vi "LabVIEW结合知识库调用本地大模型.vi"() -> ()   [LabVIEW 2023, in "LabVIEW RAG.lvlib"]
uses:
  RAG_LV_API/LabVIEW RAG.lvlib
  labview-local-model/openai_message.ctl
  labview-local-model/chat-completion req.ctl
  <vilib>/Utility/error.llb/Trim Whitespace One-Sided.vi
  labview-local-model/LabVIEW LLM.lvlib
  labview-ai-share/LabVIEW AI Base.lvlib
panel:
  in  "Manage VectorDB":bool
  in  "知识库名":string="NI-cDAQ"
  in  "Top K":u32=5
  in  "API Key":string
  in  "system prompt":string="请注意，当用户询问有关NI硬件（如cDAQ）的问题时，cDAQ-9219 与 NI-9219、\"NI 9219\" 或 \"NI-9219\" 指的是同一种硬件。" caption="System提示词"
  in  "Stream?":bool
  in  "temperature (default: 0.8)":dbl=0.8 format="%.1f"
  in  "max tokens (default: 4096)":u32=4096
  in  "Clear":bool
  in  "model URL":string="http://localhost:1234/v1"
  in  "Send":bool
  in  "Input":string="NI 9230有多少个模拟输入通道？"
  in  "选择本地模型":string(combo)
  out "error out":errorcluster
  in  "STOP":bool
  out "对话":string
  # "LabVIEW调用本地大模型"
  # "参数"
  # "知识库相关参数"
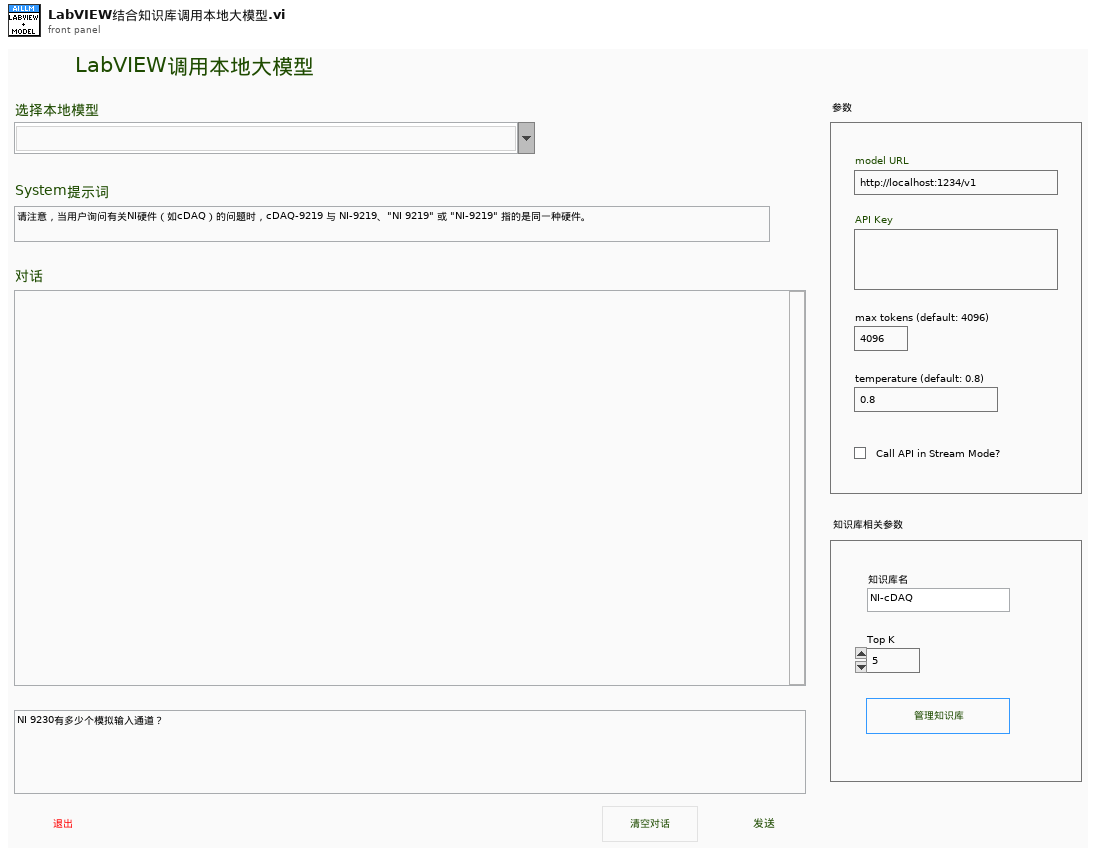
[diagram p1: front panel]
types:
  T1 = typedef "LabVIEW LLM.lvlib/openai_message.ctl" = cluster{"role":enum16{"system", "user", "assistant"}, "content":string, "reasoning":string}
  T2 = typedef "LabVIEWHTTPClient.lvlib/ClientHandle.ctl" = refnum<k1>
  T3 = typedef "LabVIEW LLM.lvlib/chat-completion req.ctl" = cluster{"model":string, "messages":T1[], "max_tokens":u32, "temperature":dbl, "stream":bool, "reasoning":cluster{"effort":enum16{"high", "medium", "low"}, "exclude":bool}}
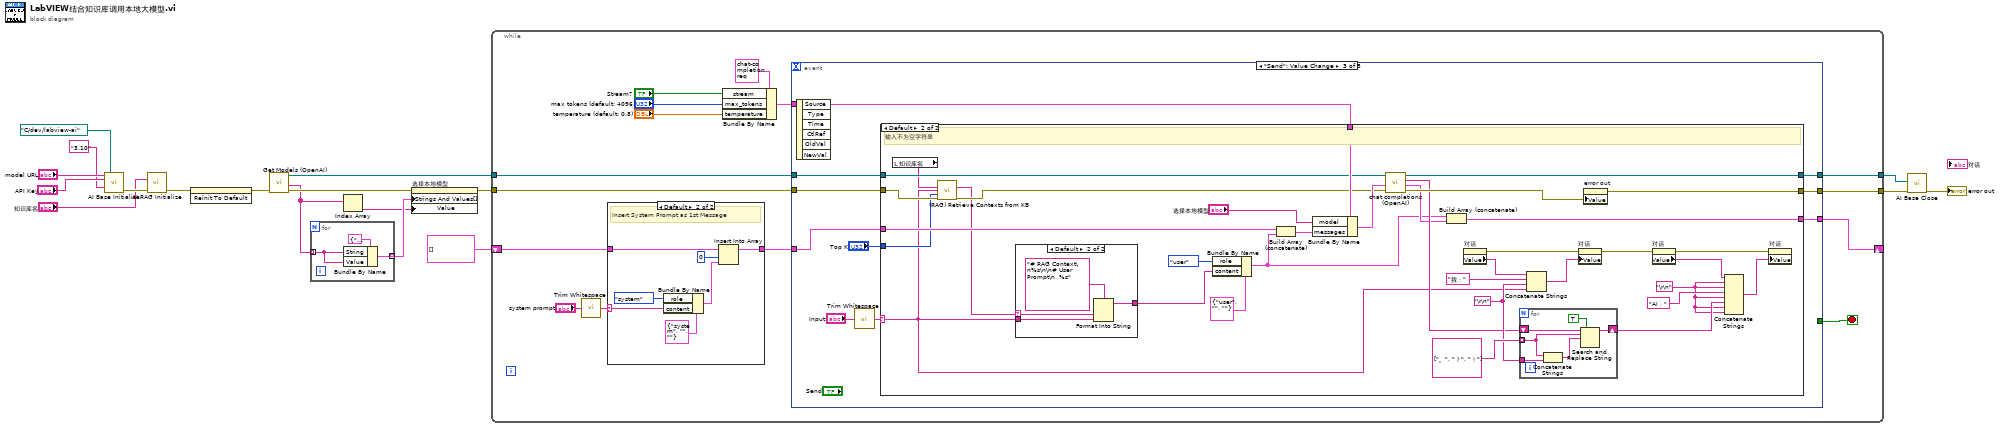
[diagram p0: block diagram]
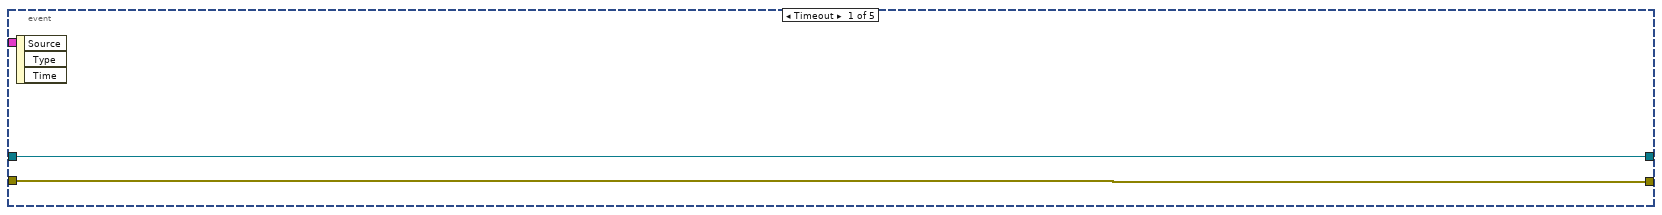
[diagram p3: hidden frame]
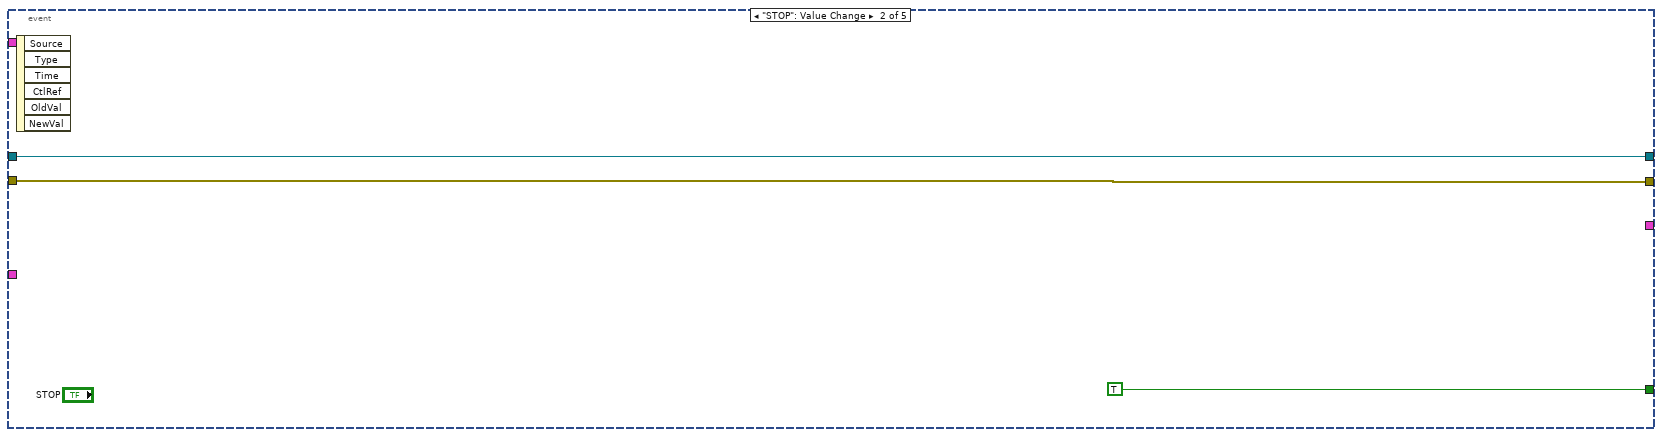
[diagram p4: hidden frame]
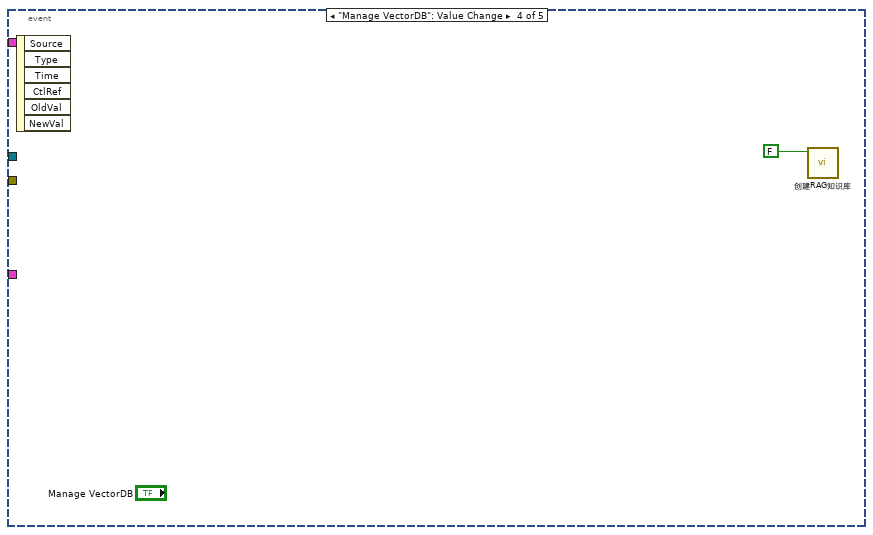
[diagram p7: hidden frame]
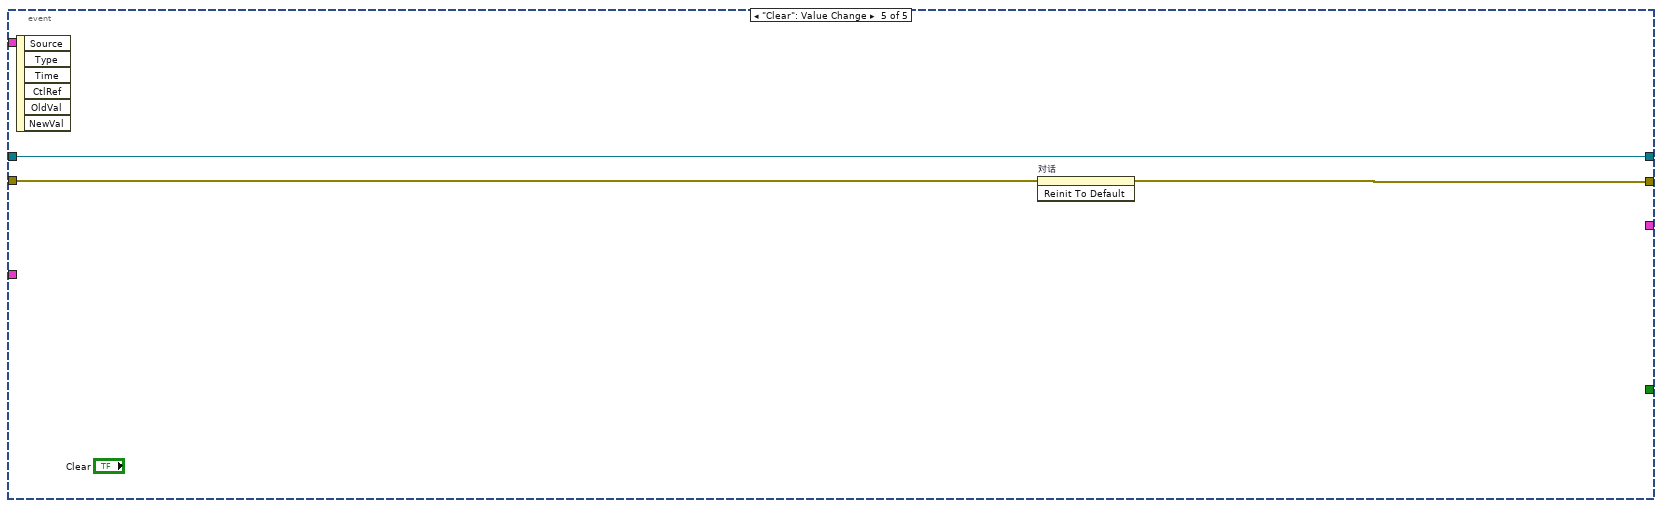
[diagram p8: hidden frame]
diagram:
  n1 = call "AI Base Initialize.vi"("OpenAI API URL"="model URL", "Python venv path"=path "C:/dev/labview-ai", "API Key"="API Key", "Python version"="3.10") -> ("error out"=w7:errorcluster)  [unwired: 9 in, 2 out]
  n2 = call "AI RAG Initialize.vi"("Knowledge Base Name"="知识库名", "error in (no error)"=w7) -> ("error out"=w4:errorcluster)  [unwired: 13 in]
  n3 = invoke on="Input" class="Str" method="Reinit To Default"(error in=w4) -> (error out=w9:errorcluster)  [unwired: 2 in, 2 out]
  n4 = call "Get Models (OpenAI).vi"("error in (no error)"=w9) -> ("error out"=w13:errorcluster, "Available Models"=w10:string[], "Refnum out"=w15:T2)  [unwired: 7 in, 1 out]
  n5 = for {
    tunnel: [w20] -> w14 mode=indexing
    tunnel: w10 -> [w19] mode=indexing
    n6 = Bundle By Name(cluster=cluster{"String":string, "Value":string} {"String"="", "Value"=""} ("Cluster"), "String"=w19, "Value"=w19) -> (w20:cluster{"String":string, "Value":string})
  }
  n7 = Index Array(array=w10) -> (element=w11:string)  [unwired: 1 in]
  n8 = property on="选择本地模型" class="CmbBox"(error in=w13, "Strings And Values[]"=w14, "Value"=w11) -> (error out=w12:errorcluster)  [unwired: 1 in, 1 out]
  n9 = while {
    tunnel: w15 -> [w35]
    tunnel: w12 -> [w34]
    tunnel: [w33] -> w18
    tunnel: [w32] -> w17
    shift-right: [w31] -> _
    shift-left: T1[] [] ("previous messages") -> [w25]
    stop <- w36 stop-if-true
    n10 = call <vilib>:"Trim Whitespace.vi"("string"="system prompt") -> ("trimmed string"=w22:string)  [unwired: 1 in]
    n11 = case shown="Default" w22 {
      selector: w22 -> [_ w44]
      tunnel: w25 -> [w37 w39]
      tunnel: [w37 w41] -> w24
      frame "" {
      }
      frame Default {
        # "Insert System Prompt as 1st Message"
        n12 = Bundle By Name(cluster=T1 {"role"=enum."system", "content"="", "reasoning"=""} ("message"), "role"=enum16{"system", "user", "assistant"}."system", "content"=w44) -> (w40:T1)
        n13 = Insert Into Array(array=w39, index=0, new element=w40) -> (w41:T1[])
      }
    }
    n14 = Bundle By Name(cluster=T3 {"model"="", "messages"=[{"role"=enum."user", "content"="", "reasoning"=""}], "max_tokens"=4096, "temperature"=0.7, "stream"=FALSE, "reasoning"={"effort"=enum."low", "exclude"=FALSE}}, "stream"="Stream?", "max_tokens"="max tokens (default: 4096)", "temperature"="temperature (default: 0.8)") -> (w30:T3)
    n15 = event shown="[2] \"Send\": Value Change" {
      selector: _ -> [_ _ _ _ _]
      dyn-events: _ -> [_ _ _ _ _]
      timeout: _ -> [_ _ _ _ _]
      tunnel: [_ TRUE _ _ _] -> w36
      tunnel: w35 -> [w46 w48 w56 _ w112]
      tunnel: w34 -> [w45 w47 w58 _ w111]
      tunnel: w30 -> [_ _ w59 _ _]
      tunnel: [w46 w48 w57 _ w112] -> w33
      tunnel: [w45 w47 w55 _ w110] -> w32
      tunnel: [_ _ w53 _ _] -> w31
      tunnel: w24 -> [_ _ w52 _ _]
      event Timeout {
        n16 = event-data() -> ()  [unwired: 1 in, 3 out]
      }
      event "STOP": Value Change {
        n17 = event-data() -> ()  [unwired: 1 in, 6 out]
      }
      event "Send": Value Change {
        n18 = event-data() -> ()  [unwired: 1 in, 6 out]
        n19 = call <vilib>:"Trim Whitespace.vi"("string"="Input") -> ("trimmed string"=w51:string)  [unwired: 1 in]
        n20 = case shown="Default" w51 {
          selector: w51 -> [_ w64]
          tunnel: w59 -> [_ w97]
          tunnel: w58 -> [w62 w69]
          tunnel: [w61 w93] -> w57
          tunnel: w56 -> [w61 w92]
          tunnel: [w62 w91] -> w55
          tunnel: [w60 w74] -> w53
          tunnel: w52 -> [w60 w72]
          tunnel: "Top K" -> [_ w65]
          frame "" {
          }
          frame Default {
            w70 = "\r\n"
            w77 = "\r\n"
            # "输入不为空字符串"
            n21 = local read "知识库名"() -> (w63:string)
            n22 = call "(RAG) Retrieve Contexts from KB.vi"("Knowledge Base Name"=w63, "RAG Query"=w64, "K"=w65, "error in"=w69) -> ("Retrieved Contexts"=w67:string, "error out"=w68:errorcluster)  [unwired: 9 in, 1 out]
            n23 = case shown="Default" w67 {
              selector: w67 -> [_ w101]
              tunnel: [w98 w100] -> w66
              tunnel: w64 -> [w98 w99]
              frame "" {
              }
              frame Default {
                n24 = Format Into String(format string="# RAG Context\n%s\n\n# User Prompt\n  %s", w101, w99) -> (resulting string=w100:string)  [unwired: 2 in, 1 out]
              }
            }
            n25 = Bundle By Name(cluster=T1 {"role"=enum."user", "content"="", "reasoning"=""} ("messages"), "role"=enum16{"system", "user", "assistant"}."user", "content"=w66) -> (w73:T1)
            n26 = Build Array (concatenate)(w72, w73) -> (w94:T1[])
            n27 = Bundle By Name(cluster=w97, "model"="选择本地模型", "messages"=w94) -> (w96:T3)
            n28 = call "chat completions (OpenAI).vi"("error in"=w68, "chat-completion req"=w96, "Refnum in"=w92) -> ("error out"=w90:errorcluster, "previous messages"=w75:T1[], "Answer content"=w76:string, "Refnum out"=w93:T2)  [unwired: 4 in, 1 out]
            n29 = Build Array (concatenate)(w73, w75) -> (w74:T1[])
            n30 = property on="对话" class="Str"() -> (error out=w89:errorcluster, "Value"=w88:string)  [unwired: 2 in, 1 out]
            n31 = for {
              tunnel: string[] ["。", "？", "！"] ("search string") -> [w106] mode=indexing
              tunnel: w77 -> [w104]
              shift-right: [w108] -> w79
              shift-left: w76 -> [w103]
              n32 = Concatenate Strings(w106, w104) -> (w105:string)
              n33 = Search and Replace String(replace all?=TRUE ("replace all? (F)"), input string=w103, search string=w106, replace string=w105) -> (result string=w108:string)  [unwired: 4 in, 3 out]
            }
            n34 = Concatenate Strings(w88, "我：" ("string"), w77, w64) -> (w87:string)
            n35 = property on="对话" class="Str"(error in=w89, "Value"=w87) -> (error out=w82:errorcluster)  [unwired: 1 in, 1 out]
            n36 = property on="error out" class="Clust (strict)"("Value"=w90) -> (error out=w91:errorcluster)  [unwired: 2 in, 1 out]
            n37 = property on="对话" class="Str"(error in=w82) -> (error out=w83:errorcluster, "Value"=w80:string)  [unwired: 1 in, 1 out]
            n38 = Concatenate Strings(w80, w70, w70, "AI：" ("string"), w70, w79, w70, w70) -> (w81:string)
            n39 = property on="对话" class="Str"(error in=w83, "Value"=w81) -> ()  [unwired: 1 in, 2 out]
          }
        }
      }
      event "Manage VectorDB": Value Change {
        n40 = event-data() -> ()  [unwired: 1 in, 6 out]
        n41 = call "创建RAG知识库.vi"("init base£"=FALSE) -> ()  [unwired: 11 in]
      }
      event "Clear": Value Change {
        n42 = event-data() -> ()  [unwired: 1 in, 6 out]
        n43 = invoke on="对话" class="Str" method="Reinit To Default"(error in=w111) -> (error out=w110:errorcluster)  [unwired: 2 in, 2 out]
      }
    }
  }
  n44 = call "AI Base Close.vi"("error in"=w17, "Http Refnum in"=w18) -> ("error out"=→"error out":errorcluster)  [unwired: 9 in]
